vi "Move Swap Probe.vi"(0 "source path":path, 5 "target path":path, 11 "error in":errorcluster) -> (4 "new path":path, 6 "cancelled":bool, 15 "error out":errorcluster)   [LabVIEW 2026]
doc: "Probe: Move outputs new path (path) and cancelled (boolean)."
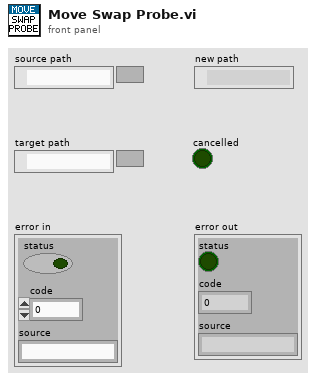
[diagram p1: front panel]
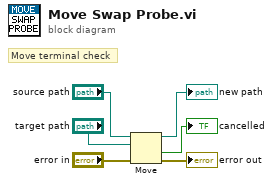
[diagram p0: block diagram]
diagram:
  # "Move terminal check"
  n1 = Move(source path="source path", error in="error in", 10:"target path") -> (error out=→"error out":errorcluster, 1:→"cancelled":bool, 3:→"new path":path)  [unwired: 2 in]
